vi "lvmcp_unbnames.vi"() -> ()   [LabVIEW 2026]
panel:
  in  "names":string[](array[string])
  out "error out":errorcluster
  in  "count":i32
  in  "reference":refnum<vi>
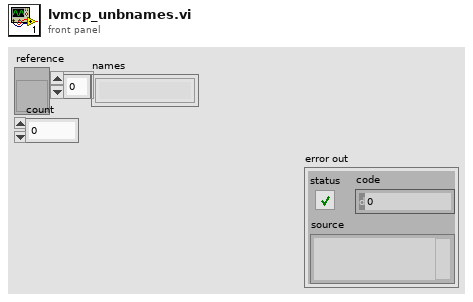
[diagram p1: front panel]
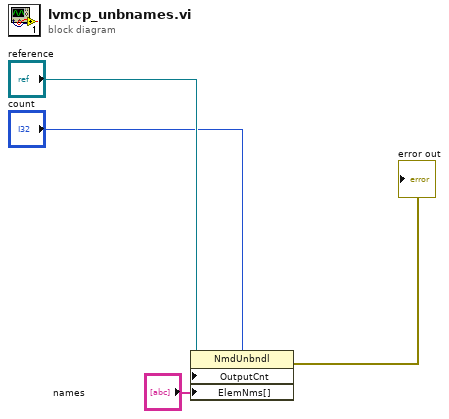
[diagram p0: block diagram]
diagram:
  n1 = property class="NmdUnbndl"(reference="reference", "OutputCnt"="count", "ElemNms[]"="names") -> (error out=→"error out":errorcluster)  [unwired: 1 in, 1 out]
